vi "ConsumeNumber.vi"(8 "error in (no error)":errorcluster, 11 "TransformTokenizer in":refnum<class "TransformTokenizer.lvclass">) -> (0 "error out":errorcluster, 3 "TransformTokenizer out":refnum<class "TransformTokenizer.lvclass">)   [LabVIEW 2019, in "TransformTokenizer.lvclass"]
uses:
  TransformTokenizer.lvclass
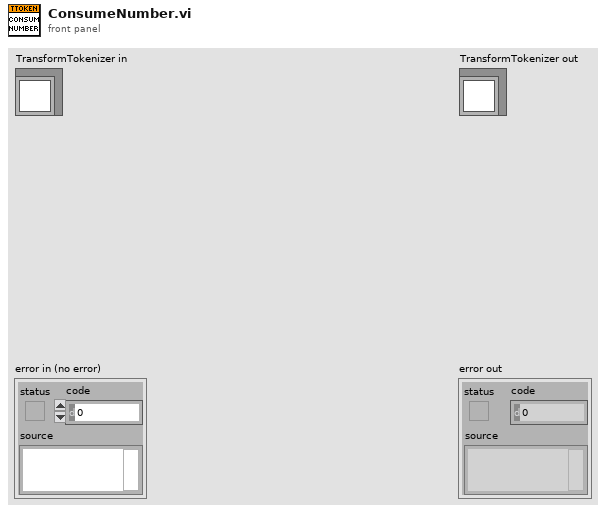
[diagram p1: front panel]
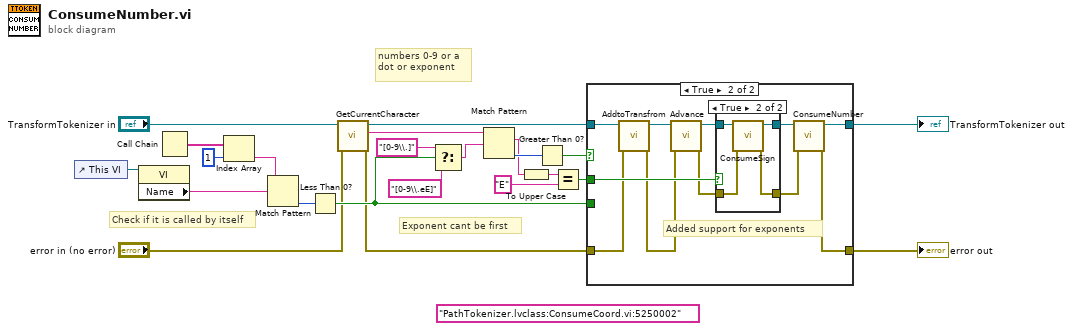
[diagram p0: block diagram]
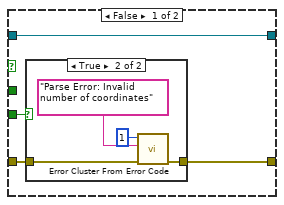
[diagram p2: hidden frame]
diagram:
  (unwired) "PathTokenizer.lvclass:ConsumeCoord.vi:5250002"
  # "Check if it is called by itself"
  # "Exponent cant be first"
  # "numbers 0-9 or a dot or exponent"
  n1 = control-ref of="This VI"() -> (w14:refnum<vi>)
  n2 = property class="VI"(reference=w14) -> ("Name"=w10:string)  [unwired: 1 in, 2 out]
  n3 = Call Chain() -> (call chain=w12:string[])
  n4 = Index Array(array=w12, index=1) -> (element=w11:string)
  n5 = Match Pattern(string=w11, regular expression=w10) -> (offset past match=w9:i32)  [unwired: 1 in, 3 out]
  n6 = Less Than 0?(x=w9) -> (x < 0?=w8:bool)
  n7 = call "GetCurrentCharacter.vi"("error in (no error)"="error in (no error)", "TransformTokenizer in"="TransformTokenizer in") -> ("error out"=w4:errorcluster, "Character"=w6:string, "TransformTokenizer out"=w5:refnum<class "TransformTokenizer.lvclass">)  [unwired: 7 in]
  n8 = Select(t="[0-9\\.]", s=w8, f="[0-9\\.eE]" ("regular expression")) -> (s? t:f=w17:string)
  n9 = Match Pattern(string=w6, regular expression=w17) -> (match substring=w21:string, offset past match=w23:i32)  [unwired: 1 in, 2 out]
  n10 = To Upper Case(1:w21) -> (0:w19:string)
  n11 = Greater Than 0?(x=w23) -> (x > 0?=w22:bool)
  n12 = Equal?(x=w19, y="E") -> (x = y?=w18:bool)
  n13 = case shown="True" w22 {
    tunnel: w5 -> [w27 w42]
    tunnel: [w27 w35] -> w3
    tunnel: w4 -> [w25 w39]
    tunnel: [w26 w34] -> w2
    tunnel: w8 -> [w24 _]
    tunnel: w18 -> [_ w43]
    frame False {
      n14 = case shown="True" w24 {
        tunnel: [w28 w32] -> w26
        tunnel: w25 -> [w28 w31]
        frame False {
        }
        frame True {
          n15 = call <vilib>:"Error Cluster From Error Code.vi"("error in (no error)"=w31, "error message (\"\")"="Parse Error: Invalid number of coordinates" ("error message (\"\")"), "error code (0)"=1) -> ("error out"=w32:errorcluster)  [unwired: 6 in]
        }
      }
    }
    frame True {
      # "Added support for exponents"
      n16 = call "AddtoTransfrom.vi"("error in (no error)"=w39, "TransformTokenizer in"=w42) -> ("error out"=w38:errorcluster, "TransformTokenizer out"=w41:refnum<class "TransformTokenizer.lvclass">)  [unwired: 8 in]
      n17 = call "Advance.vi"("error in (no error)"=w38, "TransformTokenizer in"=w41) -> ("error out"=w40:errorcluster, "TransformTokenizer out"=w37:refnum<class "TransformTokenizer.lvclass">)  [unwired: 8 in]
      n18 = case shown="True" w43 {
        tunnel: w37 -> [w45 w49]
        tunnel: [w45 w48] -> w36
        tunnel: w40 -> [w44 w47]
        tunnel: [w44 w46] -> w33
        frame False {
        }
        frame True {
          n19 = call "ConsumeSign.vi"("error in (no error)"=w47, "TransformTokenizer in"=w49) -> ("error out"=w46:errorcluster, "TransformTokenizer out"=w48:refnum<class "TransformTokenizer.lvclass">)  [unwired: 8 in]
        }
      }
      n20 = call "ConsumeNumber.vi"("error in (no error)"=w33, "TransformTokenizer in"=w36) -> ("error out"=w34:errorcluster, "TransformTokenizer out"=w35:refnum<class "TransformTokenizer.lvclass">)  [unwired: 8 in]
    }
  }
  "error out" <- w2
  "TransformTokenizer out" <- w3
